vi "Host_spb_framegr.vi"() -> ()   [LabVIEW 2018]
uses:
  <vilib>/userdefined/High Color/nirio_resource_hc.ctl
  <instrlib>/niDMM/nidmm.llb/niDMM Function.ctl
  <instrlib>/niDMM/nidmm.llb/niDMM Resolution in Digits.ctl
  <instrlib>/niDCPower/nidcpower.llb/niDCPower Measurement Type.ctl
  <instrlib>/niDMM/nidmm.llb/niDMM Configure Measurement Digits.vi
  <vilib>/FPGAPlugInAG/PXI-7953R/niLvFpga_Open_PXI-7953R.vi
  <vilib>/rvi/interface/common/dynamic/niFpgaDynamicAddResources.vi
  <vilib>/FPGAPlugInAG/Dynamic/niLvFpga_Reset_Dynamic.vi
  <vilib>/FPGAPlugInAG/Dynamic/niLvFpga_Run_Dynamic.vi
  <vilib>/Utility/error.llb/Error Cluster From Error Code.vi
  <vilib>/rvi/errors/niLvFpgaAdjustHostInterfaceError.vi
  <vilib>/FPGAPlugInAG/Dynamic/niLvFpga_Abort_Dynamic.vi
  <vilib>/rvi/interface/nirviOpenFPGA/nirviOpenFPGA.xnode
  FPGA Bitfiles/FPPZ1024M_FPGATarget_Mainspbbig_v9I9lTAMVu4.lvbitx
  <vilib>/rvi/interface/nirviMethod/nirviMethod.xnode
  <vilib>/rvi/interface/nirviReadWriteControl/nirviReadWriteControl.xnode
  <vilib>/rvi/interface/Simulation/niFpgaSimulationCallBeginRW.vi
  NiFpgaLv.dll
panel:
  in  "base path":path=path "C:/VPL/LabView_PRJ/ФППЗ_1024М/FRAMES/БОЛЬШОЙ_05"
  in  "ИМЯ":string
  in  "Запись":bool
  in  "Непрерывно":bool
  out "error out":errorcluster
  in  "Старт":bool
  out "Image":T1(plugin-control)
  in  "Interface Name":string="img0"
  in  "Фильм":bool
  in  "12":i8=12
  in  "6":i8=6
  in  "3":i8=3
  in  "Кадр":bool
  out "Промеры":i32
  in  "SIM_SEL":bool
  in  "Облучаем?":bool
  out "30_cur":dbl=0.0087480079382658 caption="Measurement" format="%.7e"
  out "28_cur":dbl=1.8081424059346318e-05 caption="Measurement" format="%.7e"
  out "18_cur":dbl=2.602551830932498e-06 caption="Measurement" format="%.7e"
  in  "NIDMM":refnum<k15>="PXI1Slot6" caption="Instrument Descriptor"
  in  "Промер токов":bool
  in  "SEL_TIME, мс":u32=100
  out "STEP":bool
  out "STEP":i32
  out "STAB_-15":bool
  out "STAB_-15":i32
  out "STAB_+15":bool
  out "STAB_+15":i32
  in  "STEP_selcur":dbl=0.20000000000000007 caption="current limit" format="%_6p"
  in  "STAB_-15_selcur":dbl=0.15 caption="current limit" format="%_6p"
  in  "STAB_+15_selcur":dbl=0.15000000000000002 caption="current limit" format="%_6p"
  in  "LOGS":path=path "C:/VPL/LabView_PRJ/ФППЗ_1024М/LOGS"
  out "Номер образца":string="0"
  in  "ТЭБ":bool
  in  "TEMP_curlim":dbl=0.3 caption="current limit" format="%_6p"
  out "TEMP_cur":dbl=0.2990767928530869 caption="measurement" format="%_6g"
  in  "TEMP, V":dbl=-10.0 caption="voltage level" format="%_6p"
  out "MUX":bool[](array[boolean])=[FALSE, FALSE, FALSE, FALSE, FALSE, TRUE, FALSE, TRUE, FALSE]
  in  "Tнак., мс":dbl=5.0
  in  "Тlight, мс":dbl=10.0
  in  "Свет":bool
  in  "Линейки":bool
  out "Configuration":bool[](array[boolean])=[FALSE, FALSE, FALSE, TRUE, TRUE, FALSE, TRUE, FALSE, FALSE]
  out "GREEN OFF":bool[](array[boolean])
  out "GREEN PGA":bool[](array[boolean])
  in  "Прошить АЦП":bool
  in  "Усиление (до 6)":u8=1
  in  "3CH/1CH":enum16{"3CH", "1CH"}(ring)=enum."1CH"
  in  "2/4 V":enum16{"2V", "4V"}(ring)
  in  "+/-":enum16{"-", "+"}(ring)=enum."+"
  in  "Смещение, до 300":dbl
  in  "LED":dbl=2.8 caption="voltage level" format="%_6p"
  in  "LED_curlim":dbl=0.012999999999999977 caption="current limit" format="%_6p"
  out "LED_cur":dbl=0.00010693387284306418 caption="measurement" format="%_6g"
  in  "REL_STEP":refnum<k15>="PXI1Slot3" caption="instrument handle"
  in  "STAB":refnum<k15>="PXI1Slot2" caption="instrument handle"
  in  "ADC":refnum<k15>="PXI1Slot4" caption="instrument handle"
  in  "Сколько строк?":i32=4096
  in  "S1_2":i16=1200
  in  "S1_1":i16=300
  in  "S2_2":i16=1500
  in  "S2_1":i16=600
  in  "S3_2":i16=950
  in  "S3_1":i16=50
  in  "Задержка после переноса строки, мкс":u16=5
  in  "ADC_2":i8=36
  in  "ADC_1":i8=12
  in  "CDS2_2":i8=44
  in  "CDS2_1":i8=32
  in  "CDS1_2":i8=24
  in  "CDS1_1":i8=8
  in  "После H, мкс":u16=5
  in  "48":i8=48
  in  "RG_2":i8=16
  in  "RG_1":i8=6
  in  "H3_2":i8=33
  in  "H3_1":i8=16
  in  "H2_2":i8=25
  in  "H2_1":i8=4
  in  "H1_2":i8=29
  in  "H1_1":i8=9
  in  "Горизонталы":i32=4096
  in  "Строка триггер":u16=1000
  in  "1800":i16=1800
  in  "REL(5V)":dbl=5.0 caption="voltage level" format="%_6p"
  in  "ADC_D(5V)":dbl=6.0 caption="voltage level" format="%_6p"
  out "STEP_cur":dbl=-1.0127765565548692e-05 caption="measurement" format="%_6g"
  out "REL_cur":dbl=4.088226600480093e-05 caption="measurement" format="%_6g"
  out "STAB_-15_cur":dbl=-5.777141877930569e-06 caption="measurement" format="%_6g"
  out "STAB_+15_cur":dbl=-5.123162671868053e-06 caption="measurement" format="%_6g"
  out "ADC_D_cur":dbl=-1.4721442871364673e-07 caption="measurement" format="%_6g"
  out "ADC_A_cur":dbl=-0.006698946789804219 caption="measurement" format="%_6g"
  in  "STEP_curlim":dbl=0.7999999999999999 caption="current limit" format="%_6p"
  in  "REL_curlim":dbl=0.30000000000000004 caption="current limit" format="%_6p"
  in  "STAB_-15_curlim":dbl=0.2 caption="current limit" format="%_6p"
  in  "STAB_+15_curlim":dbl=0.2 caption="current limit" format="%_6p"
  in  "ADC_D_curlim":dbl=0.10000000000000003 caption="current limit" format="%_6p"
  in  "ADC_A_curlim":dbl=0.1 caption="current limit" format="%_6p"
  in  "Стоп":bool
  in  "STEP(+12V)":dbl=12.0 caption="voltage level" format="%_6p"
  in  "-15V":dbl=-15.0 caption="voltage level" format="%_6p"
  in  "+15V":dbl=15.0 caption="voltage level" format="%_6p"
  in  "ADC_A(5V)":dbl=6.0 caption="voltage level" format="%_6p"
  in  "Питание":bool
  in  "resource name":T2="RIO0"
  # "РАБОТАЕМ НА ЗЕЛЕНОМ КАНАЛЕ С ВЫКЛЮЧЕННЫМИ ОСТАЛЬНЫМИ (БЕЗ ДЖАМПЕРОВ!)"
  # "0"
  # "8"
  # "0"
  # "100 дел = 3 мВ"
  # "8"
  # "0"
  # "8"
  # "0"
  # "8"
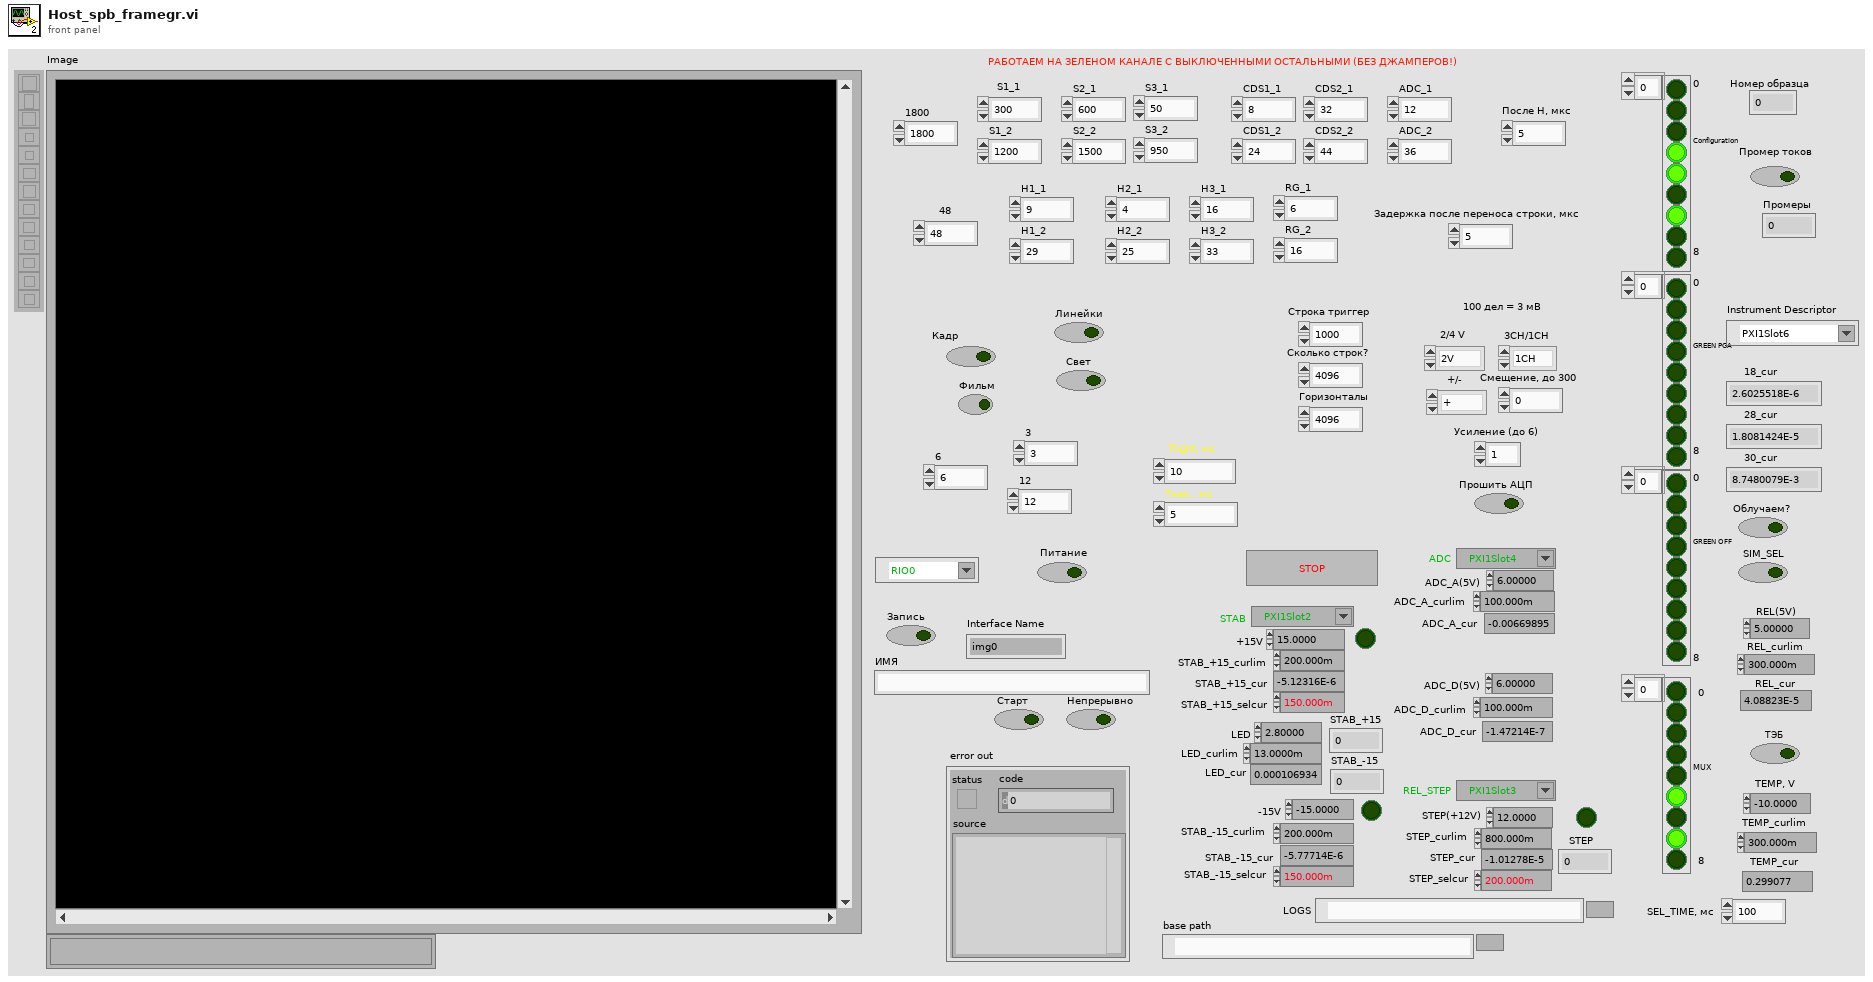
[diagram p1: front panel]
types:
  T1 = typedef "IMAQ Image.ctl" = refnum<image>
  T2 = typedef "nirio_resource_hc.ctl" = tag
  T3 = enum16{"open", "replace", "create", "open or create", "replace or create", "replace or create with confirmation"}
  T4 = typedef "niDMM Function.ctl" = enum16{"DC Volts", "AC Volts", "DC Current", "AC Current", "2-wire Resistance", "4-wire Resistance", "Diode", "Frequency", "Period", "AC Volts DC Coupled", "Capacitance", "Inductance", "Temperature"}
  T5 = typedef "niDMM Resolution in Digits.ctl" = dbl
  T6 = typedef "Image Type" = u32
  T7 = enum16{"Configuration", "MUX", "RED PGA", "GREEN PGA", "BLUE PGA", "RED OFF", "GREEN OFF", "BLUE OFF"}
  T8 = typedef "niDCPower Measurement Type.ctl" = i32
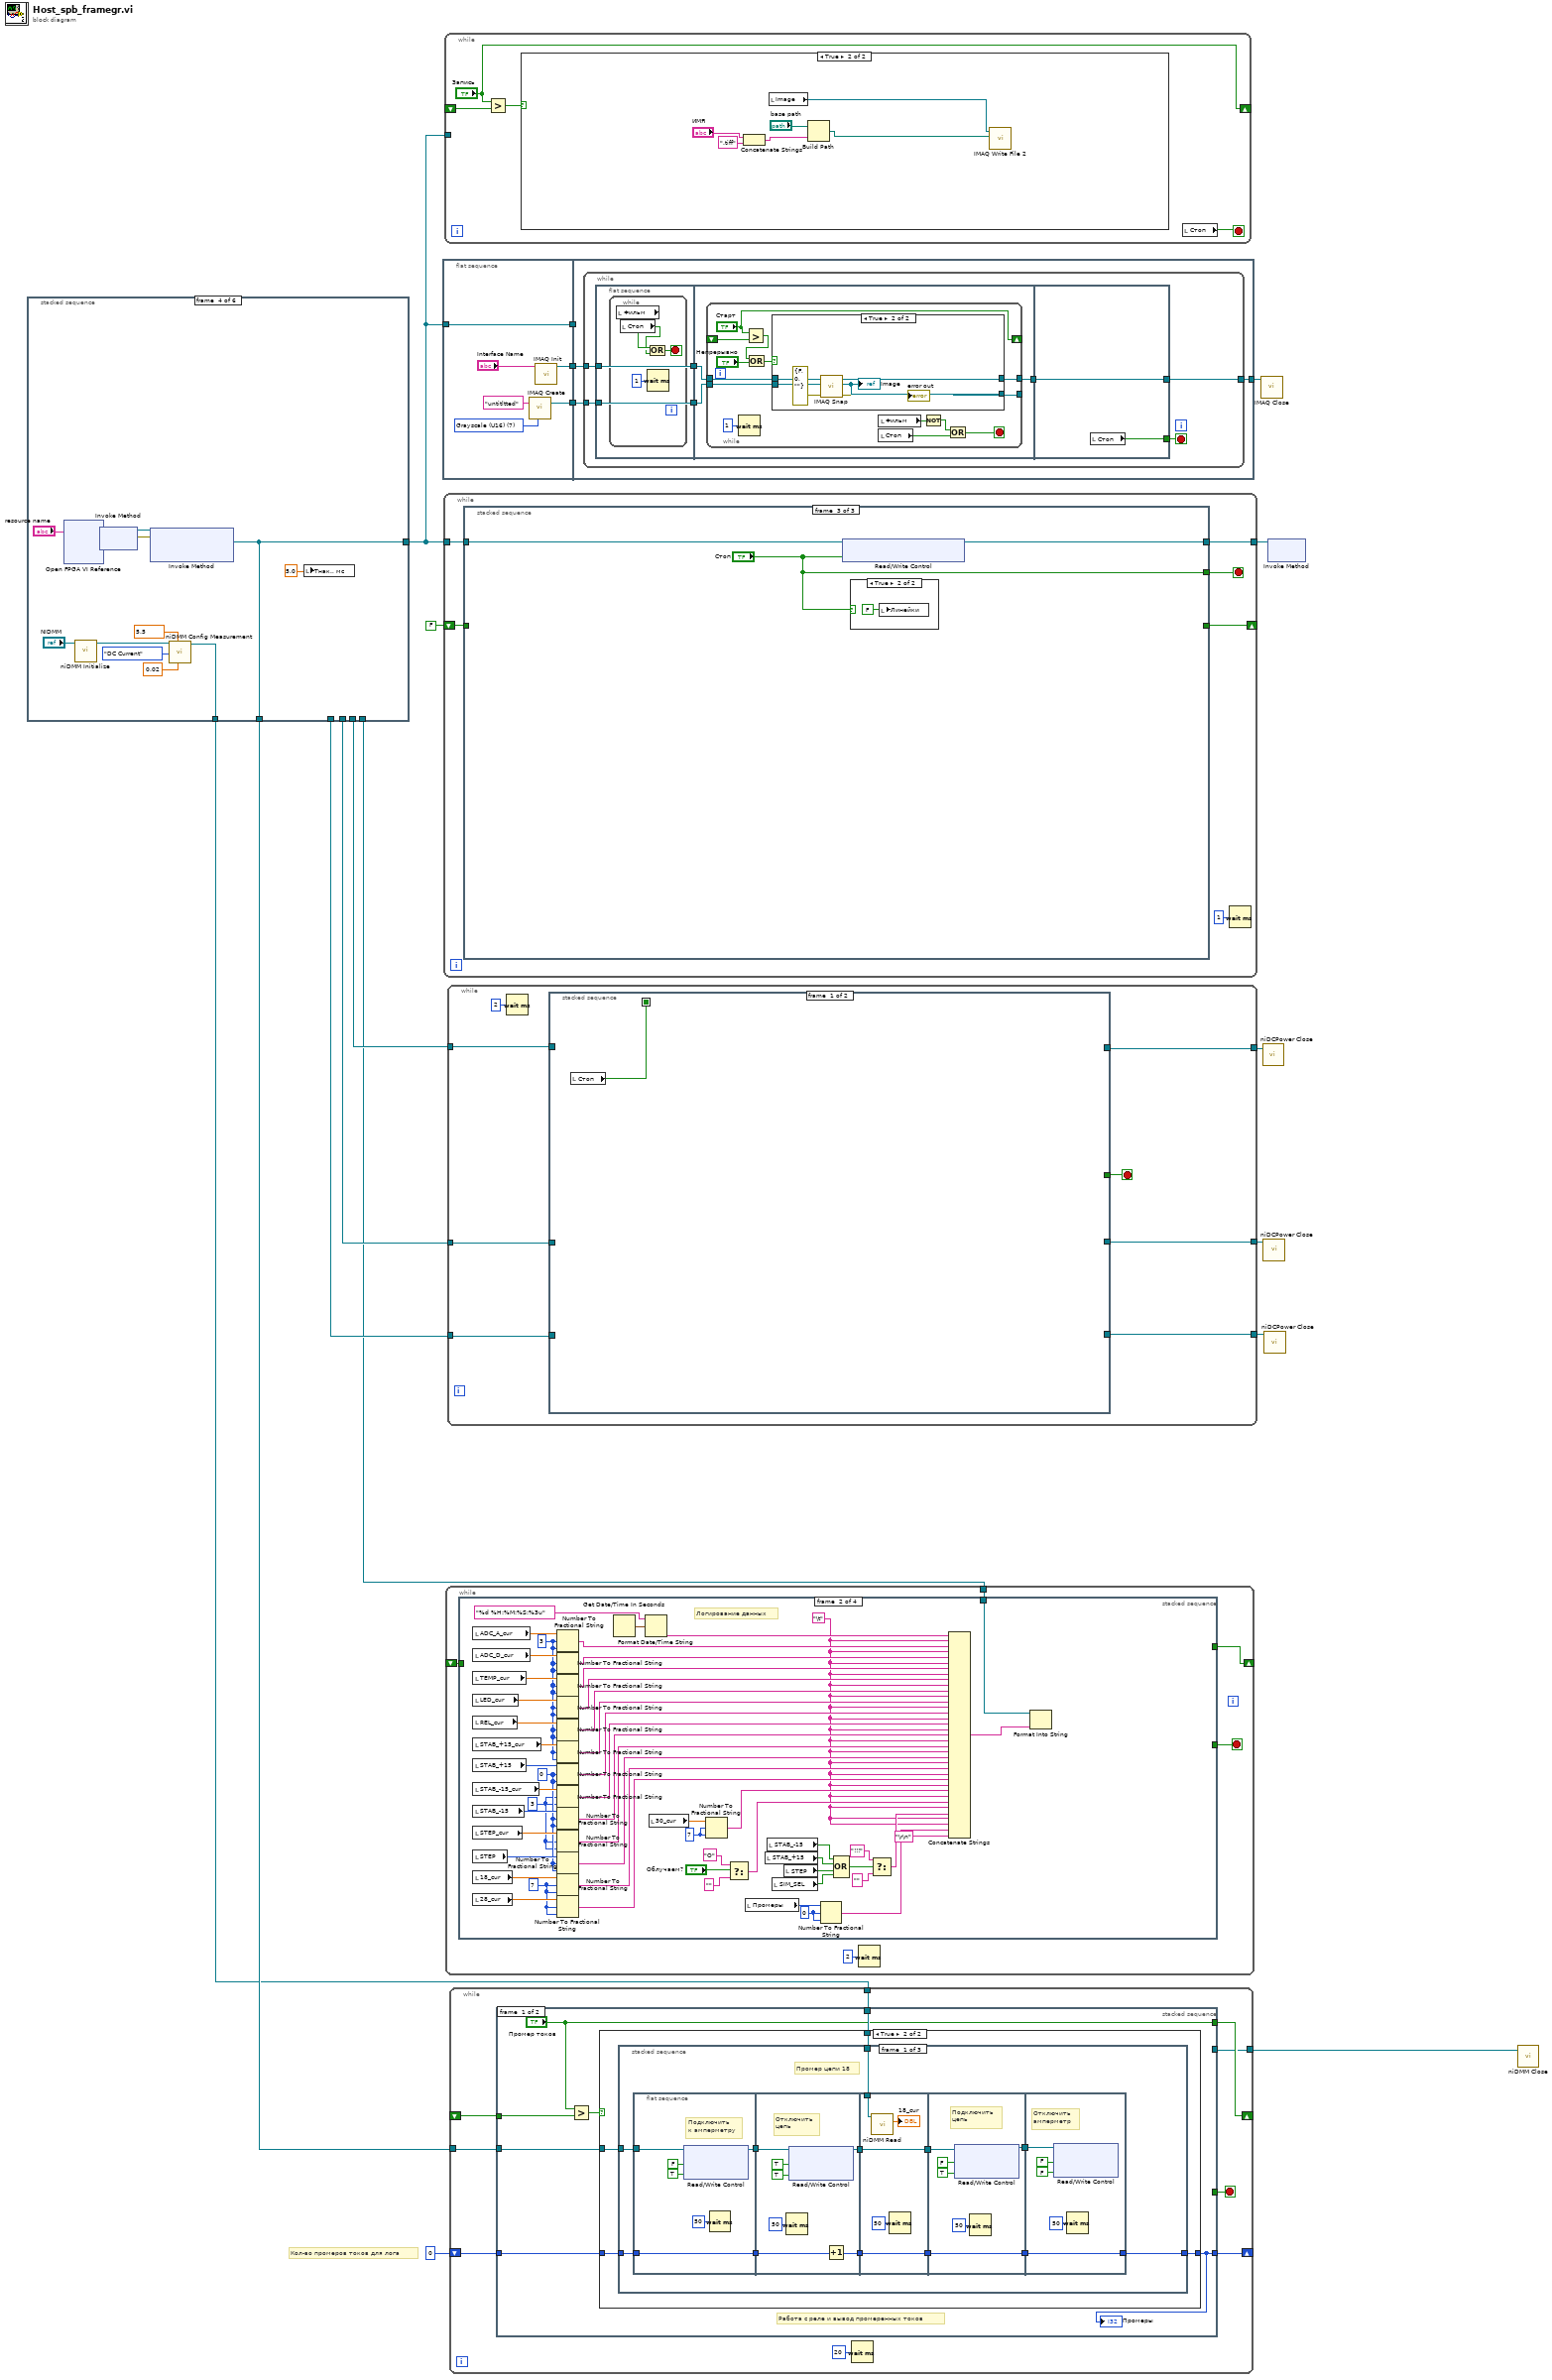
[diagram p0: block diagram]
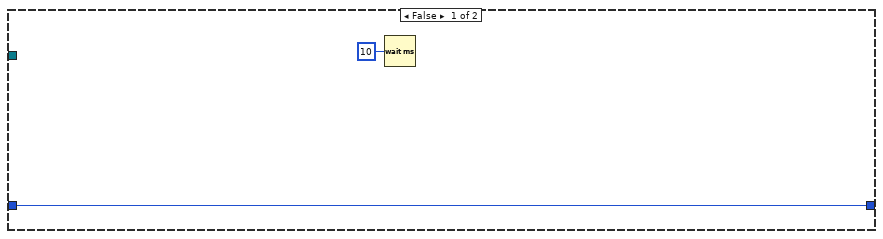
[diagram p4: hidden frame]
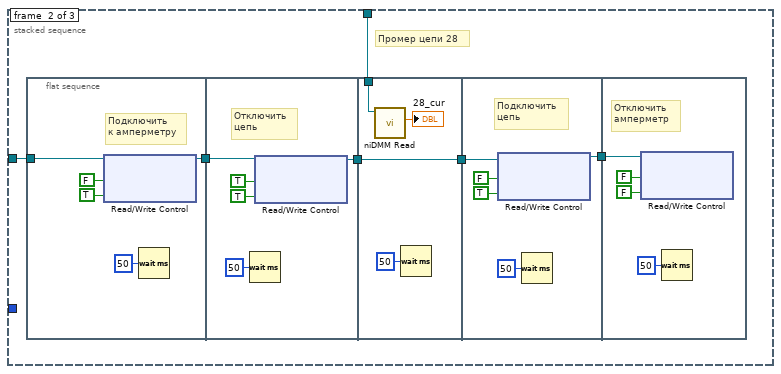
[diagram p5: hidden frame]
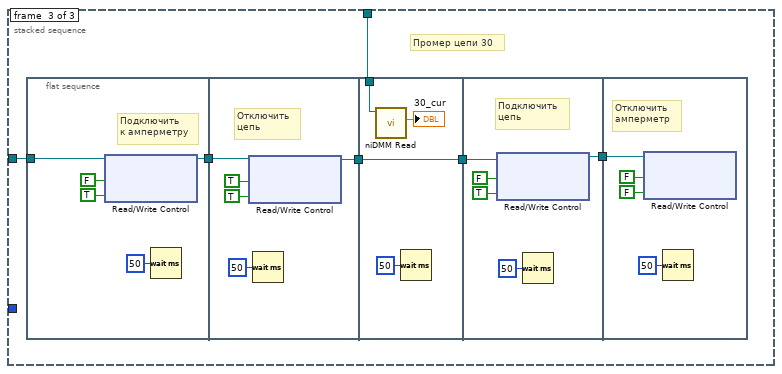
[diagram p6: hidden frame]
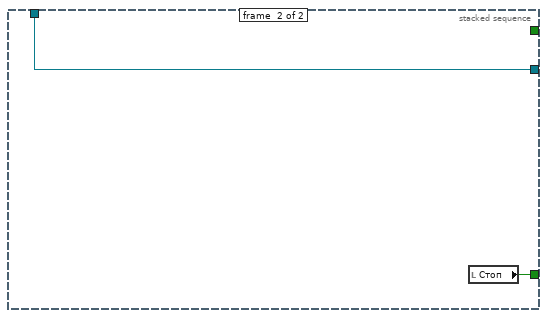
[diagram p7: hidden frame]
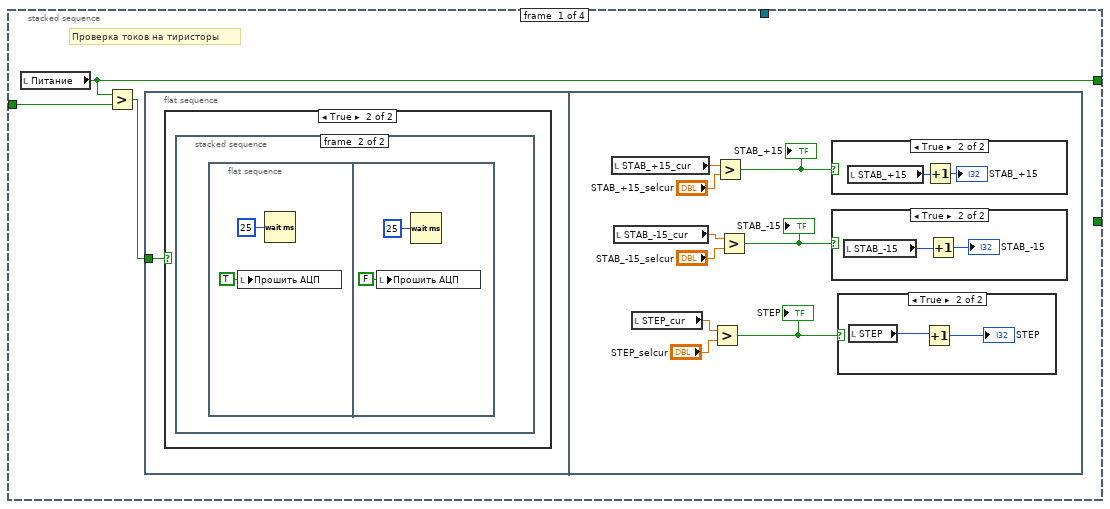
[diagram p8: hidden frame]
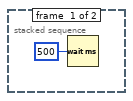
[diagram p10: hidden frame]
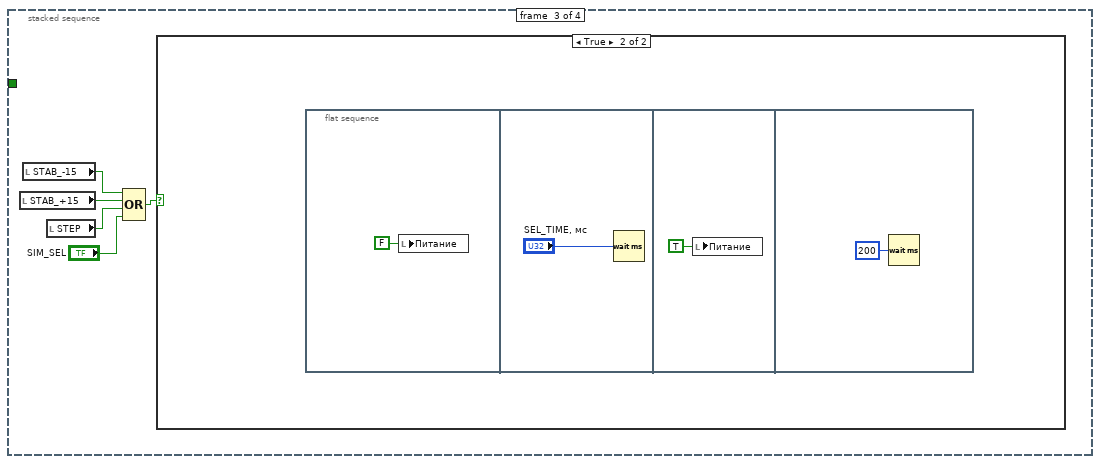
[diagram p14: hidden frame]
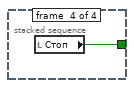
[diagram p16: hidden frame]
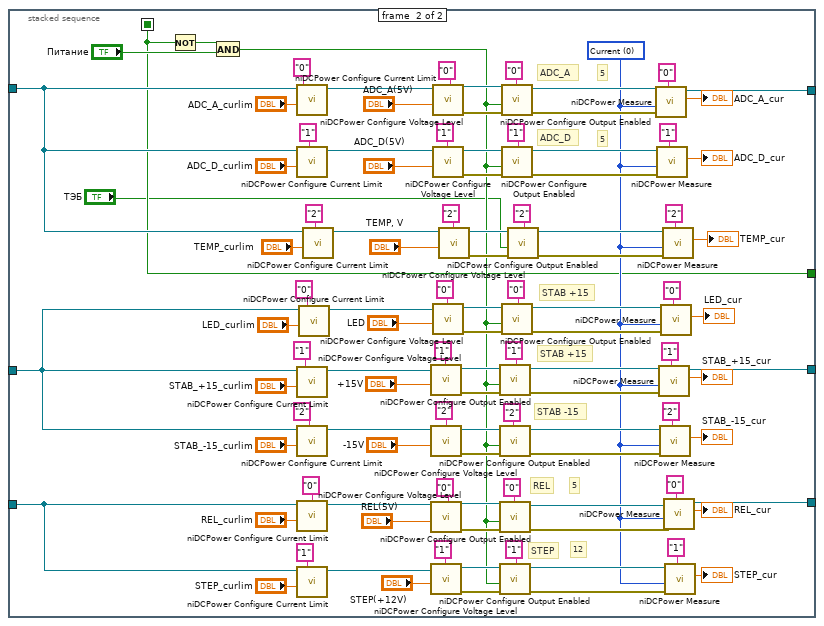
[diagram p17: hidden frame]
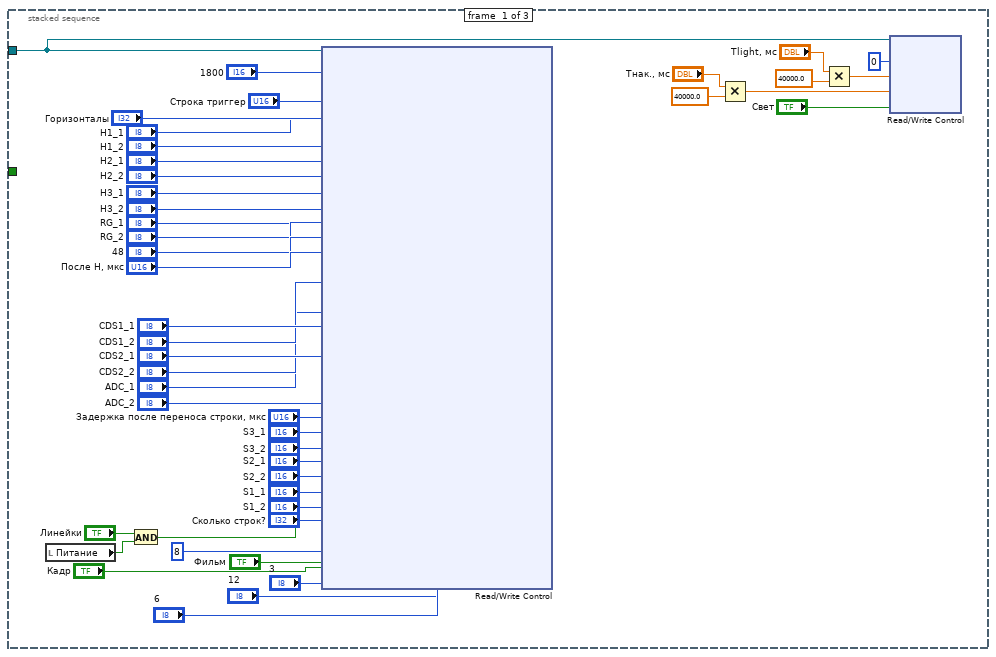
[diagram p18: hidden frame]
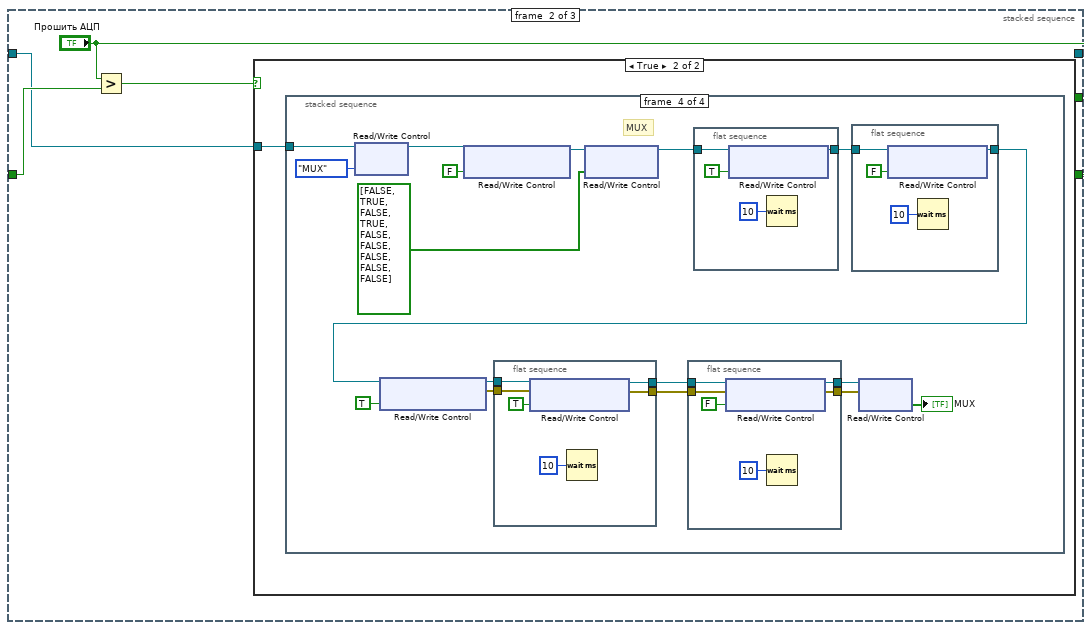
[diagram p19: hidden frame]
diagram:
  # "Кол-во промеров токов для лога"
  n1 = stacked-sequence {
    tunnel: [_ _ _ w67 _ _] -> w1
    tunnel: [_ _ _ _ w80 _] -> w18
    tunnel: [_ _ _ _ w79 _] -> w17
    tunnel: [_ _ _ _ w78 _] -> w16
    tunnel: [_ _ _ w69 _ _] -> w9
    tunnel: [_ _ _ w67 _ _] -> w10
    tunnel: [_ _ w23 _ _ _] -> w7
    frame #0 {
      n2 = call "Begin.vi"() -> ("Номер образца 2"=→"Номер образца":string)  [unwired: 11 in]
    }
    frame #1 {
      w21 = u8 0 ("Кол-во кадров")
      w20 = FALSE ("Стоп")
      # "Обнуление тиристоров"
      # "Отжатие всех кнопок управления"
      n3 = local write "STAB_+15"(w21) -> ()
      n4 = local write "STAB_-15"(w21) -> ()
      n5 = local write "STEP"(w21) -> ()
      n6 = local write "Непрерывно"(w20) -> ()
      n7 = local write "Фильм"(w20) -> ()
      n8 = local write "Стоп"(w20) -> ()
      n9 = local write "STAB_+15"(w20) -> ()
      n10 = local write "STAB_-15"(w20) -> ()
      n11 = local write "STEP"(w20) -> ()
      n12 = local write "Питание"(w20) -> ()
      n13 = local write "Линейки"(w20) -> ()
    }
    frame #2 {
      w26 = "\t"
      # "Инициализаци первой строки лога по токам"
      n14 = local read "Номер образца"() -> (w53:string)
      n15 = Build Path(base path="LOGS", name or relative path=w53) -> (appended path=w55:path)
      n16 = Get Date/Time In Seconds() -> (seconds since 1Jan1904=w48:timestamp)
      n17 = call <vilib>:"Check if File or Folder Exists.vi"("path"=w55) -> ("file or folder exists?"=w56:bool, "dup path"=w57:path)  [unwired: 8 in, 1 out]
      n18 = Format Date/Time String(time format string (%c)="%d %H.%M.%S", seconds (now)=w48) -> (date/time string=w45:string)  [unwired: 1 in]
      n19 = case shown="False" w56 {
        tunnel: w57 -> [w63 w64]
        tunnel: [w62 w64] -> w22
        frame False {
          n20 = Create Folder(path (use dialog)=w63) -> (created path=w62:path)  [unwired: 2 in, 2 out]
        }
        frame True {
        }
      }
      n21 = Concatenate Strings(w45, ".xls" ("string")) -> (w43:string)
      n22 = Build Path(base path=w22, name or relative path=w43) -> (appended path=w46:path)
      n23 = Open/Create/Replace File(file path (use dialog)=w46, operation (0:open)=T3."open or create", access (0:read/write)=enum16{"read/write", "read-only", "write-only"}."read/write") -> (refnum out=w49:refnum<file>)  [unwired: 3 in, 2 out]
      n24 = case shown="True" TRUE {
        tunnel: w49 -> [w58 w61]
        tunnel: [w58 w59] -> w42
        frame False {
        }
        frame True {
          n25 = Set File Position(refnum=w61, from (0:start)=enum16{"start", "end", "current"}."end") -> (refnum out=w59:refnum<file>)  [unwired: 2 in, 1 out]
        }
      }
      n26 = Format Into String(initial string=w42, "Time" ("input 1"), w26, "ADC_A_cur" ("input 1"), w26, "ADC_D_cur" ("input 1"), w26, "TEM_cur" ("input 1"), w26, "LED_cur" ("input 1"), w26, "RELAY_cur" ("input 1"), w26, "ST+15_cur" ("input 1"), w26, "ST+15_q" ("input 1"), w26, "ST-15_cur" ("input 1"), w26, "ST-15_q" ("input 1"), w26, "STEP_cur" ("input 1"), w26, "STEP_q" ("input 1"), w26, "18_cur" ("input 1"), w26, "28_cur" ("input 1"), w26, "30_cur" ("input 1"), w26, "Облучение" ("input 1"), "\r\n") -> (resulting string=w23:refnum<file>)  [unwired: 2 in, 1 out]
    }
    frame #3 {
      w70 = T5 5.5 items=["3 1/2"=3.5, "4 1/2"=4.5, "5 1/2"=5.5, "6 1/2"=6.5, "7 1/2"=7.5] ("Resolution in Digits")
      n27 = xnode "Open FPGA VI Reference"("resource name"="resource name") -> ("FPGA VI Reference Out"=w77:refnum<k20>, "error out"=w75:errorcluster)  [unwired: 1 in]
      n28 = call <instrlib>:"niDMM Initialize.vi"("Instrument Descriptor"="NIDMM") -> ("instrument handle out"=w72:refnum<k15>)  [unwired: 9 in, 1 out]
      n29 = xnode "Invoke Method"("FPGA VI Reference In"=w77, "error in"=w75) -> ("FPGA VI Reference Out"=w74:refnum<k20>, "error out"=w76:errorcluster)
      n30 = xnode "Invoke Method"("FPGA VI Reference In"=w74, "error in"=w76) -> ("FPGA VI Reference Out"=w67:refnum<k20>)  [unwired: 1 in, 1 out]
      n31 = call-poly <instrlib>:"niDMM Config Measurement.vi"("Range"=0.02, "Resolution in Digits"=w70, "Function"=niDMM_Function."DC Current", "instrument handle"=w72) -> ("instrument handle out"=w69:refnum<k15>)  [unwired: 6 in, 1 out]
      n32 = local write "Tнак., мс"(5.0 ("Tнак., мс")) -> ()
    }
    frame #4 {
      n33 = call <instrlib>:"niDCPower Initialize.vi"("resource name"="ADC") -> ("error out"=w90:errorcluster, "instrument handle out"=w93:refnum<k15>)  [unwired: 3 in, 6 out]
      n34 = call <instrlib>:"niDCPower Initialize.vi"("resource name"="STAB") -> ("error out"=w91:errorcluster, "instrument handle out"=w94:refnum<k15>)  [unwired: 3 in, 6 out]
      n35 = call <instrlib>:"niDCPower Initialize.vi"("resource name"="REL_STEP") -> ("error out"=w92:errorcluster, "instrument handle out"=w95:refnum<k15>)  [unwired: 3 in, 6 out]
      n36 = call <instrlib>:"niDCPower Configure Voltage Level.vi"("error in (no error)"=w90, "voltage level"=0.0, "channel name"="0,1,2", "instrument handle"=w93) -> ("instrument handle out"=w78:refnum<k15>)  [unwired: 6 in, 1 out]
      n37 = call <instrlib>:"niDCPower Configure Voltage Level.vi"("error in (no error)"=w91, "voltage level"=0.0, "channel name"="0,1,2", "instrument handle"=w94) -> ("instrument handle out"=w79:refnum<k15>)  [unwired: 6 in, 1 out]
      n38 = call <instrlib>:"niDCPower Configure Voltage Level.vi"("error in (no error)"=w92, "voltage level"=0.0, "channel name"="0,1", "instrument handle"=w95) -> ("instrument handle out"=w80:refnum<k15>)  [unwired: 6 in, 1 out]
    }
    frame #5 {
      # "Здесь надо расписать данные, которые идут в лог!"
    }
  }
  n39 = flat-sequence {
    tunnel: w1 -> [w101]
    tunnel: [w101] -> w5
    tunnel: [w97] -> w4
    tunnel: [w96] -> w3
    tunnel: w5 -> [_]
    tunnel: w4 -> [w103]
    tunnel: w3 -> [w104]
    tunnel: [w102] -> w2
    frame #0 {
      w98 = T6 7 items=["Grayscale (U8)", "Grayscale (I16)", "Grayscale (SGL)", "Complex (CSG)", "RGB (U32)", "HSL (U32)", "RGB (U64)", "Grayscale (U16)"] ("Image Type")
      n40 = call "IMAQ Create"("Image Name"="untitltted", "Image Type"=w98) -> ("New Image"=w97:T1)  [unwired: 3 in, 1 out]
      n41 = call <vilib>:"IMAQ Init.vi"("Interface Name"="Interface Name") -> ("IMAQ Session Out"=w96:refnum<k11>)  [unwired: 9 in, 1 out]
    }
    frame #1 {
      n42 = while {
        tunnel: w104 -> [w111]
        tunnel: w103 -> [w110]
        tunnel: [w109] -> w102
        stop <- w105 stop-if-true
        n43 = flat-sequence {
          tunnel: [w113] -> w108
          tunnel: w111 -> [w113]
          tunnel: [w112] -> w107
          tunnel: w110 -> [w112]
          tunnel: w108 -> [w120]
          tunnel: w107 -> [w119]
          tunnel: [w118] -> w106
          tunnel: [w144] -> w109
          tunnel: w106 -> [w144]
          tunnel: [w143] -> w105
          frame #0 {
            n44 = while {
              stop <- w117 stop-if-true
              n45 = local read "Фильм"() -> (w116:bool)
              n46 = local read "Стоп"() -> (w115:bool)
              n47 = Or(x=w116, y=w115) -> (x .or. y?=w117:bool)
              n48 = Wait (ms)(milliseconds to wait=u32 1) -> ()  [unwired: 1 out]
            }
          }
          frame #1 {
            n49 = while {
              tunnel: [w128] -> w118
              tunnel: w120 -> [w130]
              tunnel: w119 -> [w129]
              tunnel: [w127] -> _
              shift-right: ["Старт"] -> _
              shift-left: _ -> [w124]
              stop <- w131 stop-if-true
              n50 = Wait (ms)(milliseconds to wait=u32 1) -> ()  [unwired: 1 out]
              n51 = Greater?(x="Старт", y=w124) -> (0:w122:bool)
              n52 = Or(x=w122, y="Непрерывно") -> (x .or. y?=w126:bool)
              n53 = case shown="True" w126 {
                tunnel: w130 -> [w136 w142]
                tunnel: w129 -> [w135 w141]
                tunnel: [w136 w140] -> w128
                tunnel: [w135 w139] -> w127
                frame False {
                }
                frame True {
                  n54 = call <vilib>:"IMAQ Snap.vi"("error in (no error)"=errorcluster {"status"=FALSE, "code"=0, "source"=""}, "Image In"=w141, "IMAQ Session In"=w142) -> ("error out"=→"error out":errorcluster, "Image Out"=w139:T1, "IMAQ Session Out"=w140:refnum<k11>)  [unwired: 6 in]
                  "Image" <- w139
                }
              }
              n55 = local read "Фильм"() -> (w134:bool)
              n56 = local read "Стоп"() -> (w132:bool)
              n57 = Not(x=w134) -> (.not. x?=w133:bool)
              n58 = Or(x=w133, y=w132) -> (x .or. y?=w131:bool)
            }
          }
          frame #2 {
            n59 = local read "Стоп"() -> (w143:bool)
          }
        }
      }
    }
  }
  n60 = while {
    tunnel: w1 -> [w150]
    tunnel: [w148] -> w12
    shift-right: [w146] -> _
    shift-left: FALSE -> [w147]
    stop <- w149 stop-if-true
    n61 = stacked-sequence {
      tunnel: w150 -> [w156 w197 w385]
      tunnel: [_ _ "Стоп"] -> w149
      tunnel: [_ _ w384] -> w148
      tunnel: w147 -> [_ w199 _]
      tunnel: [_ "Прошить АЦП" _] -> w146
      frame #0 {
        n62 = local read "Питание"() -> (w180:bool)
        n63 = And(x="Линейки", y=w180) -> (x .and. y?=w182:bool)
        n64 = xnode "Read/Write Control"("FPGA VI Reference In"=w156, "1800"="1800", "Строка триггер"="Строка триггер", "Горизонталы"="Горизонталы", "H1_1"="H1_1", "H1_2"="H1_2", "H2_1"="H2_1", "H2_2"="H2_2", "H3_1"="H3_1", "H3_2"="H3_2", "RG_1"="RG_1", "RG_2"="RG_2", "48"="48", "После H, мкс"="После H, мкс", "CDS1_1"="CDS1_1", "CDS1_2"="CDS1_2", "CDS2_1"="CDS2_1", "CDS2_2"="CDS2_2", "ADC_1"="ADC_1", "ADC_2"="ADC_2", "Задержка после переноса строки, мкс"="Задержка после переноса строки, мкс", "S3_1"="S3_1", "S3_2"="S3_2", "S2_1"="S2_1", "S2_2"="S2_2", "S1_1"="S1_1", "S1_2"="S1_2", "Сколько строк?"="Сколько строк?", "Линейки"=w182, "8"=i8 8, "3"="3", "6"="6", "12"="12", "Кадр"="Кадр", "Фильм"="Фильм") -> ()  [unwired: 2 in, 2 out]
        n65 = Multiply(x="Tнак., мс", y=40000.0) -> (x*y=w160:dbl)
        n66 = Multiply(x="Тlight, мс", y=40000.0) -> (x*y=w158:dbl)
        n67 = xnode "Read/Write Control"("FPGA VI Reference In"=w156, "Свет от"=u32 0, "Свет до"=w158, "Задержка"=w160, "Свет"="Свет") -> ()  [unwired: 1 in, 2 out]
      }
      frame #1 {
        n68 = Greater?(x="Прошить АЦП", y=w199) -> (0:w196:bool)
        n69 = case shown="True" w196 {
          tunnel: w197 -> [_ w200]
          frame False {
          }
          frame True {
            n70 = stacked-sequence {
              tunnel: w200 -> [w225 w274 w323 w354]
              frame #0 {
                w221 = TRUE ("element")
                w222 = FALSE
                # "8"
                # "0"
                # "Configuration"
                n71 = case shown="\"3CH\", Default" "3CH/1CH" {
                  tunnel: [TRUE FALSE] -> w220
                  frame "3CH", Default {
                  }
                  frame "1CH" {
                  }
                }
                n72 = case shown="\"4V\"" "2/4 V" {
                  tunnel: [FALSE TRUE] -> w218
                  frame "2V", Default {
                  }
                  frame "4V" {
                  }
                }
                n73 = xnode "Read/Write Control"("FPGA VI Reference In"=w202, "Read(T)/Write(F)"=TRUE) -> ("FPGA VI Reference Out"=w208:refnum<k20>, "error out"=w207:errorcluster)  [unwired: 1 in]
                n74 = xnode "Read/Write Control"("FPGA VI Reference In"=w225, "Enum"=T7."Configuration") -> ("FPGA VI Reference Out"=w212:refnum<k20>)  [unwired: 1 in, 1 out]
                n75 = xnode "Read/Write Control"("FPGA VI Reference In"=w212, "Read(T)/Write(F)"=FALSE) -> ("FPGA VI Reference Out"=w210:refnum<k20>)  [unwired: 1 in, 1 out]
                n76 = Build Array(w222, w222, w222, w221, w221, w220, w221, w218, FALSE) -> (w223:bool[])
                n77 = flat-sequence {
                  tunnel: w208 -> [w237]
                  tunnel: w207 -> [w236]
                  tunnel: [w235] -> w206
                  tunnel: [w234] -> w205
                  frame #0 {
                    n78 = xnode "Read/Write Control"("FPGA VI Reference In"=w237, "error in"=w236, "Конфигурация"=TRUE) -> ("FPGA VI Reference Out"=w235:refnum<k20>, "error out"=w234:errorcluster)
                    n79 = Wait (ms)(milliseconds to wait=u32 10) -> ()  [unwired: 1 out]
                  }
                }
                n80 = Reverse 1D Array(array=w223) -> (reversed array=w215:bool[])
                n81 = xnode "Read/Write Control"("FPGA VI Reference In"=w210, "Write Data"=w215) -> ("FPGA VI Reference Out"=w214:refnum<k20>)  [unwired: 1 in, 1 out]
                n82 = flat-sequence {
                  tunnel: w206 -> [w231]
                  tunnel: w205 -> [w230]
                  tunnel: [w228] -> w204
                  tunnel: [w227] -> w203
                  frame #0 {
                    n83 = xnode "Read/Write Control"("FPGA VI Reference In"=w231, "error in"=w230, "Конфигурация"=FALSE) -> ("FPGA VI Reference Out"=w228:refnum<k20>, "error out"=w227:errorcluster)
                    n84 = Wait (ms)(milliseconds to wait=u32 10) -> ()  [unwired: 1 out]
                  }
                }
                n85 = flat-sequence {
                  tunnel: w214 -> [w245]
                  tunnel: [w243] -> w213
                  frame #0 {
                    n86 = xnode "Read/Write Control"("FPGA VI Reference In"=w245, "Конфигурация"=TRUE) -> ("FPGA VI Reference Out"=w243:refnum<k20>)  [unwired: 1 in, 1 out]
                    n87 = Wait (ms)(milliseconds to wait=u32 10) -> ()  [unwired: 1 out]
                  }
                }
                n88 = xnode "Read/Write Control"("FPGA VI Reference In"=w204, "error in"=w203) -> ("READ"=→"Configuration":bool[])  [unwired: 2 out]
                n89 = flat-sequence {
                  tunnel: w213 -> [w241]
                  tunnel: [w239] -> w202
                  frame #0 {
                    n90 = xnode "Read/Write Control"("FPGA VI Reference In"=w241, "Конфигурация"=FALSE) -> ("FPGA VI Reference Out"=w239:refnum<k20>)  [unwired: 1 in, 1 out]
                    n91 = Wait (ms)(milliseconds to wait=u32 10) -> ()  [unwired: 1 out]
                  }
                }
              }
              frame #1 {
                # "GREEN OFF"
                n92 = xnode "Read/Write Control"("FPGA VI Reference In"=w261, "Read(T)/Write(F)"=TRUE) -> ("FPGA VI Reference Out"=w272:refnum<k20>, "error out"=w271:errorcluster)  [unwired: 1 in]
                n93 = case shown="\"-\", Default" "+/-" {
                  tunnel: [TRUE FALSE] -> w252
                  frame "-", Default {
                  }
                  frame "+" {
                  }
                }
                n94 = Quotient & Remainder(x="Смещение, до 300", y=1.171875) -> (floor(x/y)=w257:dbl)  [unwired: 1 out]
                n95 = xnode "Read/Write Control"("FPGA VI Reference In"=w274, "Enum"=T7."GREEN OFF") -> ("FPGA VI Reference Out"=w265:refnum<k20>, "error out"=w264:errorcluster)  [unwired: 1 in]
                n96 = Subtract(x=w257, y=1.0) -> (x-y=w254:dbl)
                n97 = flat-sequence {
                  tunnel: w272 -> [w295]
                  tunnel: w271 -> [w294]
                  tunnel: [w293] -> w270
                  tunnel: [w292] -> w269
                  frame #0 {
                    n98 = xnode "Read/Write Control"("FPGA VI Reference In"=w295, "error in"=w294, "Конфигурация"=TRUE) -> ("FPGA VI Reference Out"=w293:refnum<k20>, "error out"=w292:errorcluster)
                    n99 = Wait (ms)(milliseconds to wait=u32 10) -> ()  [unwired: 1 out]
                  }
                }
                n100 = To Unsigned Byte Integer(number=w254) -> (unsigned 8bit integer=w253:u8)
                n101 = xnode "Read/Write Control"("FPGA VI Reference In"=w265, "error in"=w264, "Read(T)/Write(F)"=FALSE) -> ("FPGA VI Reference Out"=w263:refnum<k20>)  [unwired: 1 out]
                n102 = Number To Boolean Array(number=w253) -> (Boolean array=w251:bool[])
                n103 = Reverse 1D Array(array=w251) -> (reversed array=w250:bool[])
                n104 = Build Array (concatenate)(w252, w250) -> (w255:bool[])
                n105 = xnode "Read/Write Control"("FPGA VI Reference In"=w263, "Write Data"=w255) -> ("FPGA VI Reference Out"=w276:refnum<k20>)  [unwired: 1 in, 1 out]
                n106 = flat-sequence {
                  tunnel: w270 -> [w285]
                  tunnel: w269 -> [w284]
                  tunnel: [w282] -> w268
                  tunnel: [w281] -> w267
                  frame #0 {
                    n107 = xnode "Read/Write Control"("FPGA VI Reference In"=w285, "error in"=w284, "Конфигурация"=FALSE) -> ("FPGA VI Reference Out"=w282:refnum<k20>, "error out"=w281:errorcluster)
                    n108 = Wait (ms)(milliseconds to wait=u32 10) -> ()  [unwired: 1 out]
                  }
                }
                n109 = flat-sequence {
                  tunnel: w276 -> [w299]
                  tunnel: [w297] -> w275
                  frame #0 {
                    n110 = xnode "Read/Write Control"("FPGA VI Reference In"=w299, "Конфигурация"=TRUE) -> ("FPGA VI Reference Out"=w297:refnum<k20>)  [unwired: 1 in, 1 out]
                    n111 = Wait (ms)(milliseconds to wait=u32 10) -> ()  [unwired: 1 out]
                  }
                }
                n112 = xnode "Read/Write Control"("FPGA VI Reference In"=w268, "error in"=w267) -> ("READ"=→"GREEN OFF":bool[])  [unwired: 2 out]
                n113 = flat-sequence {
                  tunnel: w275 -> [w289]
                  tunnel: [w287] -> w261
                  frame #0 {
                    n114 = xnode "Read/Write Control"("FPGA VI Reference In"=w289, "Конфигурация"=FALSE) -> ("FPGA VI Reference Out"=w287:refnum<k20>)  [unwired: 1 in, 1 out]
                    n115 = Wait (ms)(milliseconds to wait=u32 10) -> ()  [unwired: 1 out]
                  }
                }
              }
              frame #2 {
                w309 = FALSE
                # "GREEN PGA"
                n116 = xnode "Read/Write Control"("FPGA VI Reference In"=w321, "Read(T)/Write(F)"=TRUE) -> ("FPGA VI Reference Out"=w316:refnum<k20>, "error out"=w315:errorcluster)  [unwired: 1 in]
                n117 = Decrement(x="Усиление (до 6)") -> (x-1=w301:u8)
                n118 = Multiply(x=w301, y=378) -> (x*y=w303:i32)
                n119 = Multiply(x="Усиление (до 6)", y=5) -> (x*y=w306:i32)
                n120 = xnode "Read/Write Control"("FPGA VI Reference In"=w323, "Enum"=T7."GREEN PGA") -> ("FPGA VI Reference Out"=w320:refnum<k20>)  [unwired: 1 in, 1 out]
                n121 = Divide(x=w303, y=w306) -> (x/y=w307:dbl)
                n122 = Number To Boolean Array(number=w307) -> (Boolean array=w300:bool[])
                n123 = xnode "Read/Write Control"("FPGA VI Reference In"=w320, "Read(T)/Write(F)"=FALSE) -> ("FPGA VI Reference Out"=w319:refnum<k20>)  [unwired: 1 in, 1 out]
                n124 = flat-sequence {
                  tunnel: w316 -> [w337]
                  tunnel: w315 -> [w336]
                  tunnel: [w335] -> w314
                  tunnel: [w334] -> w313
                  frame #0 {
                    n125 = xnode "Read/Write Control"("FPGA VI Reference In"=w337, "error in"=w336, "Конфигурация"=TRUE) -> ("FPGA VI Reference Out"=w335:refnum<k20>, "error out"=w334:errorcluster)
                    n126 = Wait (ms)(milliseconds to wait=u32 10) -> ()  [unwired: 1 out]
                  }
                }
                n127 = Build Array (concatenate)(w309, w309, w309, w300) -> (w308:bool[])
                n128 = xnode "Read/Write Control"("FPGA VI Reference In"=w319, "Write Data"=w308) -> ("FPGA VI Reference Out"=w322:refnum<k20>)  [unwired: 1 in, 1 out]
                n129 = flat-sequence {
                  tunnel: w314 -> [w331]
                  tunnel: w313 -> [w330]
                  tunnel: [w328] -> w312
                  tunnel: [w327] -> w311
                  frame #0 {
                    n130 = xnode "Read/Write Control"("FPGA VI Reference In"=w331, "error in"=w330, "Конфигурация"=FALSE) -> ("FPGA VI Reference Out"=w328:refnum<k20>, "error out"=w327:errorcluster)
                    n131 = Wait (ms)(milliseconds to wait=u32 10) -> ()  [unwired: 1 out]
                  }
                }
                n132 = flat-sequence {
                  tunnel: [w344] -> w324
                  tunnel: w322 -> [w343]
                  frame #0 {
                    n133 = xnode "Read/Write Control"("FPGA VI Reference In"=w343, "Конфигурация"=TRUE) -> ("FPGA VI Reference Out"=w344:refnum<k20>)  [unwired: 1 in, 1 out]
                    n134 = Wait (ms)(milliseconds to wait=u32 10) -> ()  [unwired: 1 out]
                  }
                }
                n135 = flat-sequence {
                  tunnel: w324 -> [w341]
                  tunnel: [w339] -> w321
                  frame #0 {
                    n136 = xnode "Read/Write Control"("FPGA VI Reference In"=w341, "Конфигурация"=FALSE) -> ("FPGA VI Reference Out"=w339:refnum<k20>)  [unwired: 1 in, 1 out]
                    n137 = Wait (ms)(milliseconds to wait=u32 10) -> ()  [unwired: 1 out]
                  }
                }
                n138 = xnode "Read/Write Control"("FPGA VI Reference In"=w312, "error in"=w311) -> ("READ"=→"GREEN PGA":bool[])  [unwired: 2 out]
              }
              frame #3 {
                # "MUX"
                n139 = xnode "Read/Write Control"("FPGA VI Reference In"=w354, "Enum"=T7."MUX") -> ("FPGA VI Reference Out"=w348:refnum<k20>)  [unwired: 1 in, 1 out]
                n140 = xnode "Read/Write Control"("FPGA VI Reference In"=w347, "Read(T)/Write(F)"=TRUE) -> ("FPGA VI Reference Out"=w361:refnum<k20>, "error out"=w360:errorcluster)  [unwired: 1 in]
                n141 = xnode "Read/Write Control"("FPGA VI Reference In"=w348, "Read(T)/Write(F)"=FALSE) -> ("FPGA VI Reference Out"=w350:refnum<k20>)  [unwired: 1 in, 1 out]
                n142 = flat-sequence {
                  tunnel: w361 -> [w382]
                  tunnel: w360 -> [w381]
                  tunnel: [w380] -> w359
                  tunnel: [w379] -> w358
                  frame #0 {
                    n143 = xnode "Read/Write Control"("FPGA VI Reference In"=w382, "error in"=w381, "Конфигурация"=TRUE) -> ("FPGA VI Reference Out"=w380:refnum<k20>, "error out"=w379:errorcluster)
                    n144 = Wait (ms)(milliseconds to wait=u32 10) -> ()  [unwired: 1 out]
                  }
                }
                n145 = xnode "Read/Write Control"("FPGA VI Reference In"=w350, "Write Data"=bool[] [FALSE, TRUE, FALSE, TRUE, FALSE, FALSE, FALSE, FALSE, FALSE]) -> ("FPGA VI Reference Out"=w351:refnum<k20>)  [unwired: 1 in, 1 out]
                n146 = flat-sequence {
                  tunnel: w359 -> [w376]
                  tunnel: w358 -> [w375]
                  tunnel: [w373] -> w357
                  tunnel: [w372] -> w356
                  frame #0 {
                    n147 = xnode "Read/Write Control"("FPGA VI Reference In"=w376, "error in"=w375, "Конфигурация"=FALSE) -> ("FPGA VI Reference Out"=w373:refnum<k20>, "error out"=w372:errorcluster)
                    n148 = Wait (ms)(milliseconds to wait=u32 10) -> ()  [unwired: 1 out]
                  }
                }
                n149 = flat-sequence {
                  tunnel: [w369] -> w352
                  tunnel: w351 -> [w368]
                  frame #0 {
                    n150 = xnode "Read/Write Control"("FPGA VI Reference In"=w368, "Конфигурация"=TRUE) -> ("FPGA VI Reference Out"=w369:refnum<k20>)  [unwired: 1 in, 1 out]
                    n151 = Wait (ms)(milliseconds to wait=u32 10) -> ()  [unwired: 1 out]
                  }
                }
                n152 = flat-sequence {
                  tunnel: w352 -> [w366]
                  tunnel: [w364] -> w347
                  frame #0 {
                    n153 = xnode "Read/Write Control"("FPGA VI Reference In"=w366, "Конфигурация"=FALSE) -> ("FPGA VI Reference Out"=w364:refnum<k20>)  [unwired: 1 in, 1 out]
                    n154 = Wait (ms)(milliseconds to wait=u32 10) -> ()  [unwired: 1 out]
                  }
                }
                n155 = xnode "Read/Write Control"("FPGA VI Reference In"=w357, "error in"=w356) -> ("READ"=→"MUX":bool[])  [unwired: 2 out]
              }
            }
          }
        }
      }
      frame #2 {
        n156 = xnode "Read/Write Control"("FPGA VI Reference In"=w385, "Остановка основного цикла"="Стоп") -> ("FPGA VI Reference Out"=w384:refnum<k20>)  [unwired: 1 in, 1 out]
        n157 = case shown="True" "Стоп" {
          frame False {
          }
          frame True {
            n158 = local write "Линейки"(FALSE ("Линейки")) -> ()
          }
        }
      }
    }
    n159 = Wait (ms)(milliseconds to wait=u32 1) -> ()  [unwired: 1 out]
  }
  n160 = while {
    tunnel: w1 -> [_]
    shift-right: ["Запись"] -> _
    shift-left: _ -> [w389]
    stop <- w390 stop-if-true
    n161 = Greater?(x="Запись", y=w389) -> (0:w387:bool)
    n162 = case shown="True" w387 {
      frame False {
      }
      frame True {
        n163 = Concatenate Strings("ИМЯ", ".tiff" ("string")) -> (w392:string)
        n164 = local read "Image"() -> (w395:T1)
        n165 = Build Path(base path="base path", name or relative path=w392) -> (appended path=w391:path)
        n166 = call-poly "IMAQ Write File 2"("File Path"=w391, "Image"=w395) -> ()  [unwired: 8 in, 2 out]
      }
    }
    n167 = local read "Стоп"() -> (w390:bool)
  }
  n168 = while {
    tunnel: w7 -> [w399]
    shift-right: [w397] -> _
    shift-left: _ -> [w398]
    stop <- w401 stop-if-true
    n169 = stacked-sequence {
      tunnel: [_ _ _ w490] -> w401
      tunnel: w399 -> [_ w441 _ _]
      tunnel: w398 -> [w404 _ _ _]
      tunnel: [w403 _ _ _] -> w397
      frame #0 {
        # "Проверка токов на тиристоры"
        n170 = local read "Питание"() -> (w403:bool)
        n171 = Greater?(x=w403, y=w404) -> (0:w402:bool)
        n172 = flat-sequence {
          tunnel: w402 -> [w405]
          frame #0 {
            n173 = case shown="True" w405 {
              frame False {
              }
              frame True {
                n174 = stacked-sequence {
                  frame #0 {
                    n175 = Wait (ms)(milliseconds to wait=u32 500) -> ()  [unwired: 1 out]
                  }
                  frame #1 {
                    n176 = flat-sequence {
                      frame #0 {
                        n177 = local write "Прошить АЦП"(TRUE ("Прошить АЦП")) -> ()
                        n178 = Wait (ms)(milliseconds to wait=u32 25) -> ()  [unwired: 1 out]
                      }
                      frame #1 {
                        n179 = local write "Прошить АЦП"(FALSE ("Прошить АЦП")) -> ()
                        n180 = Wait (ms)(milliseconds to wait=u32 25) -> ()  [unwired: 1 out]
                      }
                    }
                  }
                }
              }
            }
          }
          frame #1 {
            n181 = local read "STAB_+15_cur"() -> (w419:dbl)
            n182 = local read "STAB_-15_cur"() -> (w416:dbl)
            n183 = local read "STEP_cur"() -> (w413:dbl)
            n184 = Greater?(x=w413, y="STEP_selcur") -> (0:w411:bool)
            "STEP" <- w411
            n185 = Greater?(x=w419, y="STAB_+15_selcur") -> (0:w417:bool)
            "STAB_+15" <- w417
            n186 = Greater?(x=w416, y="STAB_-15_selcur") -> (0:w414:bool)
            "STAB_-15" <- w414
            n187 = case shown="True" w417 {
              frame False {
              }
              frame True {
                n188 = local read "STAB_+15"() -> (w425:i32)
                n189 = Increment(x=w425) -> (x+1=→"STAB_+15":i32)
              }
            }
            n190 = case shown="True" w414 {
              frame False {
              }
              frame True {
                n191 = local read "STAB_-15"() -> (w422:i32)
                n192 = Increment(x=w422) -> (x+1=→"STAB_-15":i32)
              }
            }
            n193 = case shown="True" w411 {
              frame False {
              }
              frame True {
                n194 = local read "STEP"() -> (w421:i32)
                n195 = Increment(x=w421) -> (x+1=→"STEP":i32)
              }
            }
          }
        }
      }
      frame #1 {
        w428 = i16 0 ("width (-)")
        w431 = i16 7 ("width (-)")
        w457 = i16 7 ("width (-)")
        w458 = i16 3 ("width (-)")
        w459 = i16 0 ("width (-)")
        w460 = i16 3 ("width (-)")
        w430 = "\t"
        # "Логирование данных"
        n196 = local read "ADC_A_cur"() -> (w477:dbl)
        n197 = local read "ADC_D_cur"() -> (w476:dbl)
        n198 = local read "TEMP_cur"() -> (w475:dbl)
        n199 = local read "LED_cur"() -> (w474:dbl)
        n200 = local read "REL_cur"() -> (w473:dbl)
        n201 = local read "STAB_+15_cur"() -> (w472:dbl)
        n202 = local read "STAB_+15"() -> (w471:i32)
        n203 = local read "STAB_-15_cur"() -> (w470:dbl)
        n204 = local read "STAB_-15"() -> (w469:i32)
        n205 = local read "STEP_cur"() -> (w468:dbl)
        n206 = local read "STEP"() -> (w467:i32)
        n207 = local read "18_cur"() -> (w466:dbl)
        n208 = local read "28_cur"() -> (w465:dbl)
        n209 = Number To Fractional String(number=w477, width (-)=w460, precision (6)=w460) -> (F-format string=w456:string)  [unwired: 1 in]
        n210 = Number To Fractional String(number=w476, width (-)=w460, precision (6)=w460) -> (F-format string=w455:string)  [unwired: 1 in]
        n211 = Number To Fractional String(number=w475, width (-)=w460, precision (6)=w460) -> (F-format string=w454:string)  [unwired: 1 in]
        n212 = Number To Fractional String(number=w474, width (-)=w460, precision (6)=w460) -> (F-format string=w453:string)  [unwired: 1 in]
        n213 = Number To Fractional String(number=w473, width (-)=w460, precision (6)=w460) -> (F-format string=w452:string)  [unwired: 1 in]
        n214 = Number To Fractional String(number=w472, width (-)=w460, precision (6)=w460) -> (F-format string=w451:string)  [unwired: 1 in]
        n215 = Number To Fractional String(number=w471, width (-)=w459, precision (6)=w459) -> (F-format string=w450:string)  [unwired: 1 in]
        n216 = Number To Fractional String(number=w470, width (-)=w458, precision (6)=w458) -> (F-format string=w449:string)  [unwired: 1 in]
        n217 = Number To Fractional String(number=w469, width (-)=w459, precision (6)=w459) -> (F-format string=w448:string)  [unwired: 1 in]
        n218 = Number To Fractional String(number=w468, width (-)=w458, precision (6)=w458) -> (F-format string=w447:string)  [unwired: 1 in]
        n219 = Number To Fractional String(number=w467, width (-)=w459, precision (6)=w459) -> (F-format string=w446:string)  [unwired: 1 in]
        n220 = Number To Fractional String(number=w466, width (-)=w431, precision (6)=w431) -> (F-format string=w445:string)  [unwired: 1 in]
        n221 = Number To Fractional String(number=w465, width (-)=w431, precision (6)=w431) -> (F-format string=w444:string)  [unwired: 1 in]
        n222 = Get Date/Time In Seconds() -> (seconds since 1Jan1904=w480:timestamp)
        n223 = Format Date/Time String(time format string (%c)="%d %H:%M:%S:%3u", seconds (now)=w480) -> (date/time string=w478:string)  [unwired: 1 in]
        n224 = local read "30_cur"() -> (w461:dbl)
        n225 = Number To Fractional String(number=w461, width (-)=w457, precision (6)=w457) -> (F-format string=w443:string)  [unwired: 1 in]
        n226 = Select(t="О", s="Облучаем?", f="") -> (s? t:f=w442:string)
        n227 = local read "Промеры"() -> (w429:i32)
        n228 = local read "STAB_+15"() -> (w439:bool)
        n229 = local read "STAB_-15"() -> (w440:bool)
        n230 = local read "SIM_SEL"() -> (w437:bool)
        n231 = local read "STEP"() -> (w438:bool)
        n232 = Number To Fractional String(number=w429, width (-)=w428, precision (6)=w428) -> (F-format string=w427:string)  [unwired: 1 in]
        n233 = Compound Arithmetic op=OR(w440, w439, w438, w437) -> (w436:bool)
        n234 = Select(t="!!!", s=w436, f="") -> (s? t:f=w432:string)
        n235 = Concatenate Strings(w478, w430, w456, w430, w455, w430, w454, w430, w453, w430, w452, w430, w451, w430, w450, w430, w449, w430, w448, w430, w447, w430, w446, w430, w445, w430, w444, w430, w443, w430, w442, w430, w432, w430, w430, w427, "\r\n") -> (w479:string)
        n236 = Format Into String(initial string=w441, w479) -> ()  [unwired: 2 in, 2 out]
      }
      frame #2 {
        n237 = local read "STAB_+15"() -> (w483:bool)
        n238 = local read "STAB_-15"() -> (w484:bool)
        n239 = local read "STEP"() -> (w482:bool)
        n240 = Compound Arithmetic op=OR(w484, w483, w482, "SIM_SEL") -> (w485:bool)
        n241 = case shown="True" w485 {
          frame False {
          }
          frame True {
            n242 = flat-sequence {
              frame #0 {
                n243 = local write "Питание"(FALSE ("Питание")) -> ()
              }
              frame #1 {
                n244 = Wait (ms)(milliseconds to wait="SEL_TIME, мс") -> ()  [unwired: 1 out]
              }
              frame #2 {
                n245 = local write "Питание"(TRUE ("Питание")) -> ()
              }
              frame #3 {
                n246 = Wait (ms)(milliseconds to wait=u32 200) -> ()  [unwired: 1 out]
              }
            }
          }
        }
      }
      frame #3 {
        n247 = local read "Стоп"() -> (w490:bool)
      }
    }
    n248 = Wait (ms)(milliseconds to wait=u32 2) -> ()  [unwired: 1 out]
  }
  n249 = while {
    tunnel: w18 -> [w498]
    tunnel: w17 -> [w493]
    tunnel: w16 -> [w492]
    tunnel: [w497] -> w15
    tunnel: [w496] -> w14
    tunnel: [w495] -> w13
    stop <- w491 stop-if-true
    n250 = Wait (ms)(milliseconds to wait=u32 2) -> ()  [unwired: 1 out]
    n251 = stacked-sequence {
      seq-local: [w499 _] -> [_ w501]
      tunnel: w498 -> [_ w535]
      tunnel: [_ w534] -> w497
      tunnel: [_ w533] -> w496
      tunnel: [_ w532] -> w495
      tunnel: w493 -> [_ w519]
      tunnel: w492 -> [_ w506]
      tunnel: [_ w501] -> w491
      frame #0 {
        n252 = local read "Стоп"() -> (w499:bool)
      }
      frame #1 {
        w505 = T8 0 items=["Current", "Voltage"] ("measurement type")
        # "STAB +15"
        # "STAB -15"
        # "STAB +15"
        # "12"
        # "STEP"
        # "REL"
        # "5"
        # "5"
        # "5"
        # "ADC_D"
        # "ADC_A"
        n253 = Not(x=w501) -> (.not. x?=w503:bool)
        n254 = And(x=w503, y="Питание") -> (x .and. y?=w504:bool)
        n255 = call <instrlib>:"niDCPower Configure Current Limit.vi"("current limit"="ADC_A_curlim", "channel name"="0", "instrument handle"=w506) -> ("instrument handle out"=w570:refnum<k15>)  [unwired: 7 in, 1 out]
        n256 = call <instrlib>:"niDCPower Configure Current Limit.vi"("current limit"="ADC_D_curlim", "channel name"="1", "instrument handle"=w506) -> ("instrument handle out"=w571:refnum<k15>)  [unwired: 7 in, 1 out]
        n257 = call <instrlib>:"niDCPower Configure Current Limit.vi"("current limit"="STAB_+15_curlim", "channel name"="1", "instrument handle"=w519) -> ("instrument handle out"=w572:refnum<k15>)  [unwired: 7 in, 1 out]
        n258 = call <instrlib>:"niDCPower Configure Current Limit.vi"("current limit"="STAB_-15_curlim", "channel name"="2", "instrument handle"=w519) -> ("instrument handle out"=w573:refnum<k15>)  [unwired: 7 in, 1 out]
        n259 = call <instrlib>:"niDCPower Configure Current Limit.vi"("current limit"="REL_curlim", "channel name"="0", "instrument handle"=w535) -> ("instrument handle out"=w574:refnum<k15>)  [unwired: 7 in, 1 out]
        n260 = call <instrlib>:"niDCPower Configure Current Limit.vi"("current limit"="STEP_curlim", "channel name"="1", "instrument handle"=w535) -> ("instrument handle out"=w575:refnum<k15>)  [unwired: 7 in, 1 out]
        n261 = call <instrlib>:"niDCPower Configure Current Limit.vi"("current limit"="LED_curlim", "channel name"="0", "instrument handle"=w519) -> ("instrument handle out"=w525:refnum<k15>)  [unwired: 7 in, 1 out]
        n262 = call <instrlib>:"niDCPower Configure Current Limit.vi"("current limit"="TEMP_curlim", "channel name"="2", "instrument handle"=w506) -> ("instrument handle out"=w513:refnum<k15>)  [unwired: 7 in, 1 out]
        n263 = call <instrlib>:"niDCPower Configure Voltage Level.vi"("voltage level"="+15V", "channel name"="1", "instrument handle"=w572) -> ("error out"=w553:errorcluster, "instrument handle out"=w550:refnum<k15>)  [unwired: 7 in]
        n264 = call <instrlib>:"niDCPower Configure Voltage Level.vi"("voltage level"="-15V", "channel name"="2", "instrument handle"=w573) -> ("error out"=w552:errorcluster, "instrument handle out"=w551:refnum<k15>)  [unwired: 7 in]
        n265 = call <instrlib>:"niDCPower Configure Voltage Level.vi"("voltage level"="REL(5V)", "channel name"="0", "instrument handle"=w574) -> ("error out"=w562:errorcluster, "instrument handle out"=w565:refnum<k15>)  [unwired: 7 in]
        n266 = call <instrlib>:"niDCPower Configure Voltage Level.vi"("voltage level"="STEP(+12V)", "channel name"="1", "instrument handle"=w575) -> ("error out"=w563:errorcluster, "instrument handle out"=w564:refnum<k15>)  [unwired: 7 in]
        n267 = call <instrlib>:"niDCPower Configure Voltage Level.vi"("voltage level"="ADC_A(5V)", "channel name"="0", "instrument handle"=w570) -> ("error out"=w540:errorcluster, "instrument handle out"=w543:refnum<k15>)  [unwired: 7 in]
        n268 = call <instrlib>:"niDCPower Configure Voltage Level.vi"("voltage level"="ADC_D(5V)", "channel name"="1", "instrument handle"=w571) -> ("error out"=w541:errorcluster, "instrument handle out"=w542:refnum<k15>)  [unwired: 7 in]
        n269 = call <instrlib>:"niDCPower Configure Voltage Level.vi"("voltage level"="LED", "channel name"="0", "instrument handle"=w525) -> ("error out"=w529:errorcluster, "instrument handle out"=w530:refnum<k15>)  [unwired: 7 in]
        n270 = call <instrlib>:"niDCPower Configure Voltage Level.vi"("voltage level"="TEMP, V", "channel name"="2", "instrument handle"=w513) -> ("error out"=w516:errorcluster, "instrument handle out"=w515:refnum<k15>)  [unwired: 7 in]
        n271 = call <instrlib>:"niDCPower Configure Output Enabled.vi"("error in (no error)"=w553, "output enabled"=w504, "channel name"="1", "instrument handle"=w550) -> ("error out"=w599:errorcluster, "instrument handle out"=w592:refnum<k15>)  [unwired: 6 in]
        n272 = call <instrlib>:"niDCPower Configure Output Enabled.vi"("error in (no error)"=w552, "output enabled"=w504, "channel name"="2", "instrument handle"=w551) -> ("error out"=w594:errorcluster, "instrument handle out"=w593:refnum<k15>)  [unwired: 6 in]
        n273 = call <instrlib>:"niDCPower Configure Output Enabled.vi"("error in (no error)"=w562, "output enabled"=w504, "channel name"="0", "instrument handle"=w565) -> ("error out"=w596:errorcluster, "instrument handle out"=w595:refnum<k15>)  [unwired: 6 in]
        n274 = call <instrlib>:"niDCPower Configure Output Enabled.vi"("error in (no error)"=w563, "output enabled"=w504, "channel name"="1", "instrument handle"=w564) -> ("error out"=w597:errorcluster, "instrument handle out"=w598:refnum<k15>)  [unwired: 6 in]
        n275 = call <instrlib>:"niDCPower Configure Output Enabled.vi"("error in (no error)"=w540, "output enabled"=w504, "channel name"="0", "instrument handle"=w543) -> ("error out"=w583:errorcluster, "instrument handle out"=w582:refnum<k15>)  [unwired: 6 in]
        n276 = call <instrlib>:"niDCPower Configure Output Enabled.vi"("error in (no error)"=w541, "output enabled"=w504, "channel name"="1", "instrument handle"=w542) -> ("error out"=w584:errorcluster, "instrument handle out"=w585:refnum<k15>)  [unwired: 6 in]
        n277 = call <instrlib>:"niDCPower Configure Output Enabled.vi"("error in (no error)"=w529, "output enabled"=w504, "channel name"="0", "instrument handle"=w530) -> ("error out"=w521:errorcluster, "instrument handle out"=w522:refnum<k15>)  [unwired: 6 in]
        n278 = call <instrlib>:"niDCPower Configure Output Enabled.vi"("error in (no error)"=w516, "output enabled"="ТЭБ", "channel name"="2", "instrument handle"=w515) -> ("error out"=w511:errorcluster, "instrument handle out"=w510:refnum<k15>)  [unwired: 6 in]
        n279 = call <instrlib>:"niDCPower Measure.vi"("error in (no error)"=w583, "measurement type"=w505, "channel name"="0", "instrument handle"=w582) -> ("measurement"=→"ADC_A_cur":dbl, "instrument handle out"=w534:refnum<k15>)  [unwired: 5 in, 1 out]
        n280 = call <instrlib>:"niDCPower Measure.vi"("error in (no error)"=w584, "measurement type"=w505, "channel name"="1", "instrument handle"=w585) -> ("measurement"=→"ADC_D_cur":dbl)  [unwired: 5 in, 2 out]
        n281 = call <instrlib>:"niDCPower Measure.vi"("error in (no error)"=w599, "measurement type"=w505, "channel name"="1", "instrument handle"=w592) -> ("measurement"=→"STAB_+15_cur":dbl, "instrument handle out"=w533:refnum<k15>)  [unwired: 5 in, 1 out]
        n282 = call <instrlib>:"niDCPower Measure.vi"("error in (no error)"=w594, "measurement type"=w505, "channel name"="2", "instrument handle"=w593) -> ("measurement"=→"STAB_-15_cur":dbl)  [unwired: 5 in, 2 out]
        n283 = call <instrlib>:"niDCPower Measure.vi"("error in (no error)"=w521, "measurement type"=w505, "channel name"="0", "instrument handle"=w522) -> ("measurement"=→"LED_cur":dbl)  [unwired: 5 in, 2 out]
        n284 = call <instrlib>:"niDCPower Measure.vi"("error in (no error)"=w511, "measurement type"=w505, "channel name"="2", "instrument handle"=w510) -> ("measurement"=→"TEMP_cur":dbl)  [unwired: 5 in, 2 out]
        n285 = call <instrlib>:"niDCPower Measure.vi"("error in (no error)"=w596, "measurement type"=w505, "channel name"="0", "instrument handle"=w595) -> ("measurement"=→"REL_cur":dbl, "instrument handle out"=w532:refnum<k15>)  [unwired: 5 in, 1 out]
        n286 = call <instrlib>:"niDCPower Measure.vi"("error in (no error)"=w597, "measurement type"=w505, "channel name"="1", "instrument handle"=w598) -> ("measurement"=→"STEP_cur":dbl)  [unwired: 5 in, 2 out]
      }
    }
  }
  n287 = while {
    tunnel: w10 -> [w616]
    tunnel: w9 -> [w615]
    shift-right: [w613] -> _
    shift-left: _ -> [w614]
    tunnel: [w612] -> w8
    shift-right: [w608] -> _
    shift-left: 0 -> [w609]
    stop <- w611 stop-if-true
    n288 = stacked-sequence {
      tunnel: w616 -> [w622 _]
      tunnel: w615 -> [w621 w730]
      tunnel: w614 -> [w620 _]
      tunnel: ["Промер токов" _] -> w613
      tunnel: [_ w730] -> w612
      tunnel: [_ w729] -> w611
      tunnel: w609 -> [w618 _]
      tunnel: [w617 _] -> w608
      frame #0 {
        # "Работа с реле и вывод промеренных токов"
        n289 = Greater?(x="Промер токов", y=w620) -> (0:w623:bool)
        n290 = case shown="True" w623 {
          tunnel: w622 -> [_ w629]
          tunnel: w621 -> [_ w628]
          tunnel: w618 -> [w624 w627]
          tunnel: [w624 w626] -> w617
          frame False {
            n291 = Wait (ms)(milliseconds to wait=u32 10) -> ()  [unwired: 1 out]
          }
          frame True {
            n292 = stacked-sequence {
              tunnel: w629 -> [w641 w676 w705]
              tunnel: w628 -> [w640 w675 w704]
              tunnel: w627 -> [w635 _ _]
              tunnel: [w633 _ _] -> w626
              frame #0 {
                # "Промер цепи 18"
                n293 = flat-sequence {
                  tunnel: w641 -> [w647]
                  tunnel: [w646] -> w639
                  tunnel: w635 -> [w642]
                  tunnel: [w642] -> w634
                  tunnel: w639 -> [w654]
                  tunnel: [w653] -> w638
                  tunnel: w634 -> [w649]
                  tunnel: [w648] -> w630
                  tunnel: w640 -> [w659]
                  tunnel: w638 -> [w657]
                  tunnel: [w657] -> w637
                  tunnel: [w655] -> w631
                  tunnel: w630 -> [w655]
                  tunnel: w637 -> [w665]
                  tunnel: [w663] -> w636
                  tunnel: [w660] -> w632
                  tunnel: w631 -> [w660]
                  tunnel: w636 -> [w670]
                  tunnel: [w666] -> w633
                  tunnel: w632 -> [w666]
                  frame #0 {
                    # "Подключить \nк амперметру"
                    n294 = xnode "Read/Write Control"("FPGA VI Reference In"=w647, "RELAY_18_IN1"=FALSE, "RELAY_18_IN2"=TRUE) -> ("FPGA VI Reference Out"=w646:refnum<k20>)  [unwired: 1 in, 1 out]
                    n295 = Wait (ms)(milliseconds to wait=u32 50) -> ()  [unwired: 1 out]
                  }
                  frame #1 {
                    # "Отключить\nцепь"
                    n296 = Wait (ms)(milliseconds to wait=u32 50) -> ()  [unwired: 1 out]
                    n297 = xnode "Read/Write Control"("FPGA VI Reference In"=w654, "RELAY_18_IN1"=TRUE, "RELAY_18_IN2"=TRUE) -> ("FPGA VI Reference Out"=w653:refnum<k20>)  [unwired: 1 in, 1 out]
                    n298 = Increment(x=w649) -> (x+1=w648:i32)
                  }
                  frame #2 {
                    n299 = call <instrlib>:"niDMM Read.vi"("instrument handle"=w659) -> ("Measurement"=→"18_cur":dbl)  [unwired: 8 in, 2 out]
                    n300 = Wait (ms)(milliseconds to wait=u32 50) -> ()  [unwired: 1 out]
                  }
                  frame #3 {
                    # "Подключить\nцепь"
                    n301 = xnode "Read/Write Control"("FPGA VI Reference In"=w665, "RELAY_18_IN1"=FALSE, "RELAY_18_IN2"=TRUE) -> ("FPGA VI Reference Out"=w663:refnum<k20>)  [unwired: 1 in, 1 out]
                    n302 = Wait (ms)(milliseconds to wait=u32 50) -> ()  [unwired: 1 out]
                  }
                  frame #4 {
                    # "Отключить \nамперметр"
                    n303 = xnode "Read/Write Control"("FPGA VI Reference In"=w670, "RELAY_18_IN1"=FALSE, "RELAY_18_IN2"=FALSE) -> ()  [unwired: 1 in, 2 out]
                    n304 = Wait (ms)(milliseconds to wait=u32 50) -> ()  [unwired: 1 out]
                  }
                }
              }
              frame #1 {
                # "Промер цепи 28"
                n305 = flat-sequence {
                  tunnel: w676 -> [w681]
                  tunnel: [w680] -> w674
                  tunnel: w674 -> [w686]
                  tunnel: [w685] -> w673
                  tunnel: w675 -> [w690]
                  tunnel: w673 -> [w688]
                  tunnel: [w688] -> w672
                  tunnel: w672 -> [w695]
                  tunnel: [w693] -> w671
                  tunnel: w671 -> [w699]
                  frame #0 {
                    # "Подключить \nк амперметру"
                    n306 = xnode "Read/Write Control"("FPGA VI Reference In"=w681, "RELAY_28_IN1"=FALSE, "RELAY_28_IN2"=TRUE) -> ("FPGA VI Reference Out"=w680:refnum<k20>)  [unwired: 1 in, 1 out]
                    n307 = Wait (ms)(milliseconds to wait=u32 50) -> ()  [unwired: 1 out]
                  }
                  frame #1 {
                    # "Отключить\nцепь"
                    n308 = Wait (ms)(milliseconds to wait=u32 50) -> ()  [unwired: 1 out]
                    n309 = xnode "Read/Write Control"("FPGA VI Reference In"=w686, "RELAY_28_IN1"=TRUE, "RELAY_28_IN2"=TRUE) -> ("FPGA VI Reference Out"=w685:refnum<k20>)  [unwired: 1 in, 1 out]
                  }
                  frame #2 {
                    n310 = call <instrlib>:"niDMM Read.vi"("instrument handle"=w690) -> ("Measurement"=→"28_cur":dbl)  [unwired: 8 in, 2 out]
                    n311 = Wait (ms)(milliseconds to wait=u32 50) -> ()  [unwired: 1 out]
                  }
                  frame #3 {
                    # "Подключить\nцепь"
                    n312 = xnode "Read/Write Control"("FPGA VI Reference In"=w695, "RELAY_28_IN1"=FALSE, "RELAY_28_IN2"=TRUE) -> ("FPGA VI Reference Out"=w693:refnum<k20>)  [unwired: 1 in, 1 out]
                    n313 = Wait (ms)(milliseconds to wait=u32 50) -> ()  [unwired: 1 out]
                  }
                  frame #4 {
                    # "Отключить \nамперметр"
                    n314 = xnode "Read/Write Control"("FPGA VI Reference In"=w699, "RELAY_28_IN1"=FALSE, "RELAY_28_IN2"=FALSE) -> ()  [unwired: 1 in, 2 out]
                    n315 = Wait (ms)(milliseconds to wait=u32 50) -> ()  [unwired: 1 out]
                  }
                }
              }
              frame #2 {
                # "Промер цепи 30"
                n316 = flat-sequence {
                  tunnel: w705 -> [w710]
                  tunnel: [w709] -> w703
                  tunnel: w703 -> [w715]
                  tunnel: [w714] -> w702
                  tunnel: w704 -> [w719]
                  tunnel: w702 -> [w717]
                  tunnel: [w717] -> w701
                  tunnel: w701 -> [w724]
                  tunnel: [w722] -> w700
                  tunnel: w700 -> [w728]
                  frame #0 {
                    # "Подключить \nк амперметру"
                    n317 = xnode "Read/Write Control"("FPGA VI Reference In"=w710, "RELAY_30_IN1"=FALSE, "RELAY_30_IN2"=TRUE) -> ("FPGA VI Reference Out"=w709:refnum<k20>)  [unwired: 1 in, 1 out]
                    n318 = Wait (ms)(milliseconds to wait=u32 50) -> ()  [unwired: 1 out]
                  }
                  frame #1 {
                    # "Отключить\nцепь"
                    n319 = xnode "Read/Write Control"("FPGA VI Reference In"=w715, "RELAY_30_IN1"=TRUE, "RELAY_30_IN2"=TRUE) -> ("FPGA VI Reference Out"=w714:refnum<k20>)  [unwired: 1 in, 1 out]
                    n320 = Wait (ms)(milliseconds to wait=u32 50) -> ()  [unwired: 1 out]
                  }
                  frame #2 {
                    n321 = call <instrlib>:"niDMM Read.vi"("instrument handle"=w719) -> ("Measurement"=→"30_cur":dbl)  [unwired: 8 in, 2 out]
                    n322 = Wait (ms)(milliseconds to wait=u32 50) -> ()  [unwired: 1 out]
                  }
                  frame #3 {
                    # "Подключить\nцепь"
                    n323 = xnode "Read/Write Control"("FPGA VI Reference In"=w724, "RELAY_30_IN1"=FALSE, "RELAY_30_IN2"=TRUE) -> ("FPGA VI Reference Out"=w722:refnum<k20>)  [unwired: 1 in, 1 out]
                    n324 = Wait (ms)(milliseconds to wait=u32 50) -> ()  [unwired: 1 out]
                  }
                  frame #4 {
                    # "Отключить \nамперметр"
                    n325 = xnode "Read/Write Control"("FPGA VI Reference In"=w728, "RELAY_30_IN1"=FALSE, "RELAY_30_IN2"=FALSE) -> ()  [unwired: 1 in, 2 out]
                    n326 = Wait (ms)(milliseconds to wait=u32 50) -> ()  [unwired: 1 out]
                  }
                }
              }
            }
          }
        }
        "Промеры" <- w617
      }
      frame #1 {
        n327 = local read "Стоп"() -> (w729:bool)
      }
    }
    n328 = Wait (ms)(milliseconds to wait=u32 20) -> ()  [unwired: 1 out]
  }
  n329 = call <vilib>:"IMAQ Close.vi"("IMAQ Session In"=w2) -> ()  [unwired: 10 in, 1 out]
  n330 = call <instrlib>:"niDCPower Close.vi"("instrument handle"=w15) -> ()  [unwired: 10 in, 1 out]
  n331 = call <instrlib>:"niDCPower Close.vi"("instrument handle"=w14) -> ()  [unwired: 10 in, 1 out]
  n332 = call <instrlib>:"niDCPower Close.vi"("instrument handle"=w13) -> ()  [unwired: 10 in, 1 out]
  n333 = xnode "Invoke Method"("FPGA VI Reference In"=w12) -> ()  [unwired: 1 in, 2 out]
  n334 = call <instrlib>:"niDMM Close.vi"("instrument handle"=w8) -> ()  [unwired: 10 in, 1 out]
